vi "FuncVI-XYGraph.vi"(5 "InstanceRef":T2, 9 "arg list":T1[](array[typedef])) -> (0 "error out":bool, 3 "result":T1)   [LabVIEW 2021]
doc: "::: CalcExpress Toolkit :::\nCopyright (c) 2000-2026 Konstantin Shifershteyn. All rights reserved."
uses:
  cetypes.llb/CalcExpress Function Argument Info.ctl
  cetypes.llb/CalcExpress Instance RefNum.ctl
panel:
  in  "max arg num":i32=7
  in  "min arg num":i32
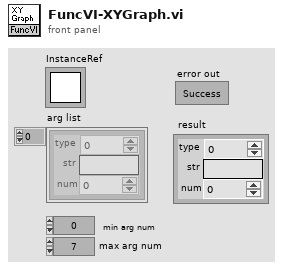
[diagram p1: front panel]
types:
  T1 = typedef "CalcExpress Function Argument Info.ctl" = cluster{"type":u32, "str":string, "num":dbl}
  T2 = typedef "CalcExpress Instance RefNum.ctl" = refnum<k1>
  T3 = cluster{"index":i32, "type":enum8{"String", "DBL Number", "identifier", "1D Array of DBL", "2D Array of DBL", "CDB Number", "1D Array of CDB", "2D Array of CDB", "Unknown data type"}, "default num":dbl, "default str":string}[]
  T4 = cluster{"data type":enum32{"String", "DBL Number", "identifier", "1D Array of DBL", "2D Array of DBL", "CDB Number", "1D Array of CDB", "2D Array of CDB", "1D Array of String", "2D Array of String", "Unknown data type"}, "str":string, "num":dbl}
  T5 = cluster{"index":i32, "type":enum8{"String", "DBL Number", "identifier", "1D Array of DBL", "2D Array of DBL", "CDB Number", "1D Array of CDB", "2D Array of CDB", "Unknown data type"}, "default num":dbl, "default str":string}
  T6 = cluster{i32, "Sine Wave":dbl[], "Sine Wave":dbl[], "str":string}
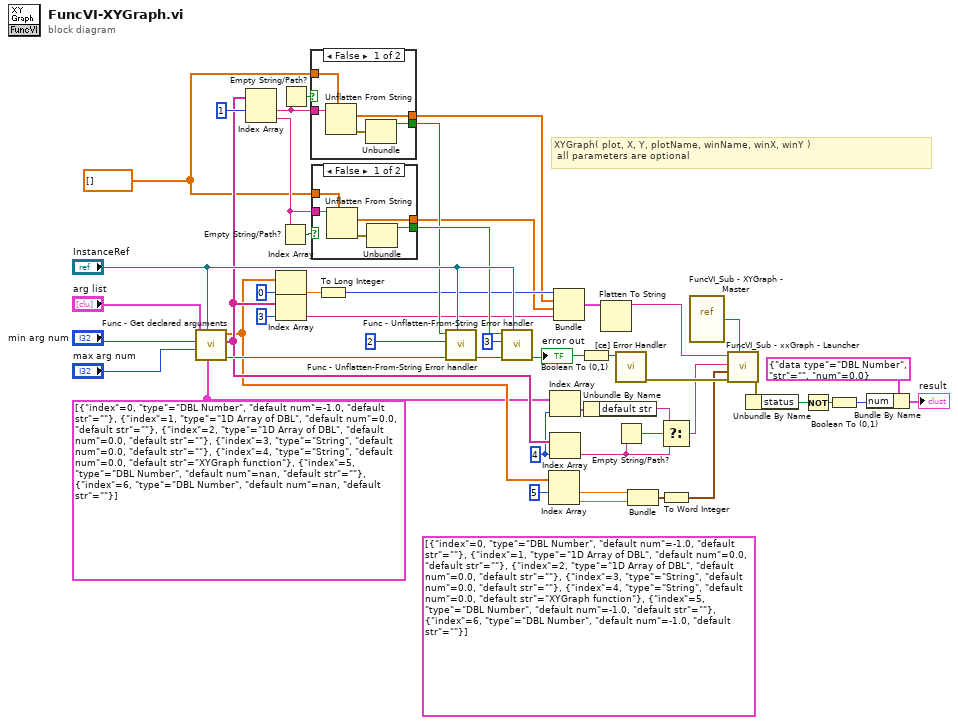
[diagram p0: block diagram]
diagram:
  (unwired) T3 [{"index"=0, "type"=enum."DBL Number", "default num"=-1.0, "default str"=""}, {"index"=1, "type"=enum."1D Array of DBL", "default num"=0.0, "default str"=""}, {"index"=2, "type"=enum."1D Array of DBL", "default num"=0.0, "default str"=""}, {"index"=3, "type"=enum."String", "default num"=0.0, "default str"=""}, {"index"=4, "type"=enum."String", "default num"=0.0, "default str"="XYGraph function"}, {"index"=5, "type"=enum."DBL Number", "default num"=-1.0, "default str"=""}, {"index"=6, "type"=enum."DBL Number", "default num"=-1.0, "default str"=""}] ("args descriptors")
  w7 = 4
  w2 = dbl[] [] ("Sine Wave")
  w6 = T3 [{"index"=0, "type"=enum."DBL Number", "default num"=-1.0, "default str"=""}, {"index"=1, "type"=enum."1D Array of DBL", "default num"=0.0, "default str"=""}, {"index"=2, "type"=enum."1D Array of DBL", "default num"=0.0, "default str"=""}, {"index"=3, "type"=enum."String", "default num"=0.0, "default str"=""}, {"index"=4, "type"=enum."String", "default num"=0.0, "default str"="XYGraph function"}, {"index"=5, "type"=enum."DBL Number", "default num"=nan, "default str"=""}, {"index"=6, "type"=enum."DBL Number", "default num"=nan, "default str"=""}] ("args descriptors")
  # "XYGraph( plot, X, Y, plotName, winName, winX, winY ) \n all parameters are optional"
  n1 = call "Func - Get declared arguments.vi"("arg descriptors"=w6, "InstanceRef"="InstanceRef", "max arg num"="max arg num", "min arg num"="min arg num", "arg list"="arg list") -> ("error out"=w41:bool, "str list"=w14:string[], "num list"=w13:dbl[])  [unwired: 3 in, 1 out]
  n2 = Index Array(array=w14, index #1=1) -> (element #1=w46:string, element #2=w3:string)  [unwired: 1 in]
  n3 = Index Array(array=w13, index=0) -> (element=w43:dbl)
  n4 = Index Array(array=w14, index=3) -> (element=w31:string)
  n5 = Empty String/Path?(string/path=w3) -> (empty?=w42:bool)
  n6 = Empty String/Path?(string/path=w46) -> (empty?=w47:bool)
  n7 = case shown="False" w47 {
    tunnel: [w54 _] -> w37
    tunnel: [w53 w55] -> w30
    tunnel: w2 -> [w52 w55]
    tunnel: w46 -> [w51 _]
    frame False {
      n8 = Unflatten From String(type=w52, binary string=w51) -> (value=w53:dbl[], error out=w50:errorcluster)  [unwired: 3 in, 1 out]
      n9 = Unbundle(w50) -> ("status"=w54:bool)  [unwired: 2 out]
    }
    frame True {
    }
  }
  n10 = case shown="False" w42 {
    tunnel: [w60 _] -> w38
    tunnel: [w59 w61] -> w29
    tunnel: w2 -> [w58 w61]
    tunnel: w3 -> [w57 _]
    frame False {
      n11 = Unflatten From String(type=w58, binary string=w57) -> (value=w59:dbl[], error out=w56:errorcluster)  [unwired: 3 in, 1 out]
      n12 = Unbundle(w56) -> ("status"=w60:bool)  [unwired: 2 out]
    }
    frame True {
    }
  }
  n13 = To Long Integer(number=w43) -> (32bit integer=w32:i32)
  n14 = call "Func - Unflatten-From-String Error handler.vi"("InstanceRef"="InstanceRef", "error in"=w41, "argument number"=2, "Unflatten Error status"=w37) -> ("error out"=w40:bool)  [unwired: 5 in]
  n15 = call "Func - Unflatten-From-String Error handler.vi"("InstanceRef"="InstanceRef", "error in"=w40, "argument number"=3, "Unflatten Error status"=w38) -> ("error out"=w27:bool)  [unwired: 5 in]
  "error out" <- w27
  n16 = Index Array(array=w13, index #1=5) -> (element #1=w16:dbl, element #2=w15:dbl)  [unwired: 1 in]
  n17 = Index Array(array=w6, index=w7) -> (element=w8:T5)
  n18 = Index Array(array=w14, index=w7) -> (element=w5:string)
  n19 = Bundle(w32, "Sine Wave"=w30, "Sine Wave"=w29, "str"=w31) -> (w25:T6)  [unwired: 1 in]
  n20 = Boolean To (0,1)(Boolean=w27) -> (0, 1=w28:i16)
  n21 = Unbundle By Name(w8) -> ("default str"=w9:string)
  n22 = Flatten To String(anything=w25) -> (data string=w24:string)  [unwired: 3 in, 2 out]
  n23 = call "[ce] Error Handler.vi"("error code"=w28) -> ("error out"=w26:errorcluster)  [unwired: 9 in, 1 out]
  n24 = Empty String/Path?(string/path=w5) -> (empty?=w10:bool)
  n25 = Bundle("str"=w16, "str"=w15) -> (w12:cluster{"str":dbl, "str":dbl})  [unwired: 1 in]
  n26 = Select(t=w9, s=w10, f=w5) -> (s? t:f=w4:string)
  n27 = To Word Integer(number=w12) -> (16bit integer=w11:cluster{"str":i16, "str":i16})
  n28 = vi-ref "FuncVI_Sub - XYGraph - Master.vi"() -> (w1:refnum<vi>)
  n29 = call "FuncVI_Sub - xxGraph - Launcher.vi"("Master VI Refnum"=w1, "error in"=w26, "left-top corner"=w11, "win name"=w4, "data"=w24) -> ("error out"=w18:errorcluster)  [unwired: 6 in]
  n30 = Unbundle By Name(w18) -> ("status"=w20:bool)
  n31 = Not(x=w20) -> (.not. x?=w23:bool)
  n32 = Boolean To (0,1)(Boolean=w23) -> (0, 1=w21:i16)
  n33 = Bundle By Name(cluster=T4 {"data type"=enum."DBL Number", "str"="", "num"=0.0} ("opd info"), "num"=w21) -> (→"result":T4)
